vi "Write opened.vi"(8 "error in (no error)":errorcluster, 10 "opened":bool, 11 "ZM-CP-communication_protocol in":refnum<class "ZM-CP-communication_protocol.lvclass">) -> (0 "error out":errorcluster, 3 "ZM-CP-communication_protocol out":refnum<class "ZM-CP-communication_protocol.lvclass">)   [LabVIEW 2020, in "ZM-CP-communication_protocol.lvlib" / "ZM-CP-communication_protocol.lvclass"]
doc: "Writes one field of this class's private data. Generated by lvai_create_accessors from the class private data control."
uses:
  ZM-CP-communication_protocol.lvclass
  ZM-CP-communication_protocol.lvclass/ZM-CP-communication_protocol.ctl
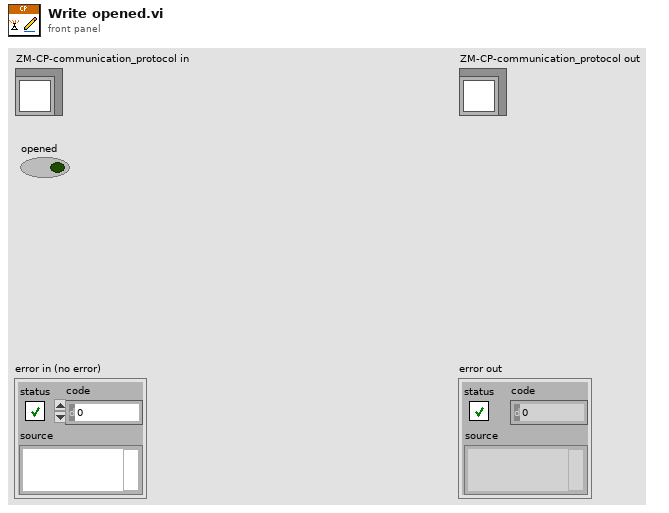
[diagram p1: front panel]
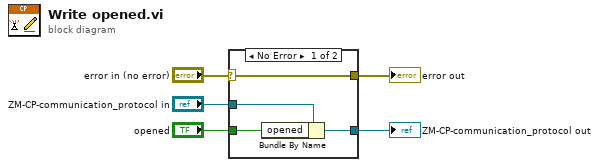
[diagram p0: block diagram]
diagram:
  n1 = case shown="No Error" "error in (no error)" {
    selector: "error in (no error)" -> [w9 w10]
    tunnel: [w9 w10] -> w4
    tunnel: [w7 w11] -> w2
    tunnel: "ZM-CP-communication_protocol in" -> [w8 w11]
    tunnel: "opened" -> [w6 _]
    frame No Error {
      n2 = Bundle By Name(cluster=w8, "opened"=w6) -> (w7:refnum<class "ZM-CP-communication_protocol.lvclass">)
    }
    frame Error {
    }
  }
  "error out" <- w4
  "ZM-CP-communication_protocol out" <- w2
